vi "getFont.vi"(0 "reference":refnum<class "Graphics.lvclass">, 5 "error in (no error)":errorcluster) -> (14 "reference out":refnum<class "Graphics.lvclass">, 15 "fontType":T2=enum."Application Font", 16 "font":T1, 17 "size":i16, 19 "error out":errorcluster)   [LabVIEW 2020, in "Graphics.lvclass"]
doc: "Get font info"
uses:
  <resource>/Framework/Providers/Open_GDS/UML/Graphics_class/Graphics.lvclass
  <resource>/Framework/Providers/Open_GDS/UML/Graphics_class/LvFontType.ctl
  <resource>/Framework/Providers/Open_GDS/UML/Graphics_class/FontType.ctl
panel:
  # "Always set\nVI Server class\nto current VI. Do not\nconnect this control\nto the connector pane.\n(Tip!: Just drag\nand drop the icon\ninto the refnum)"
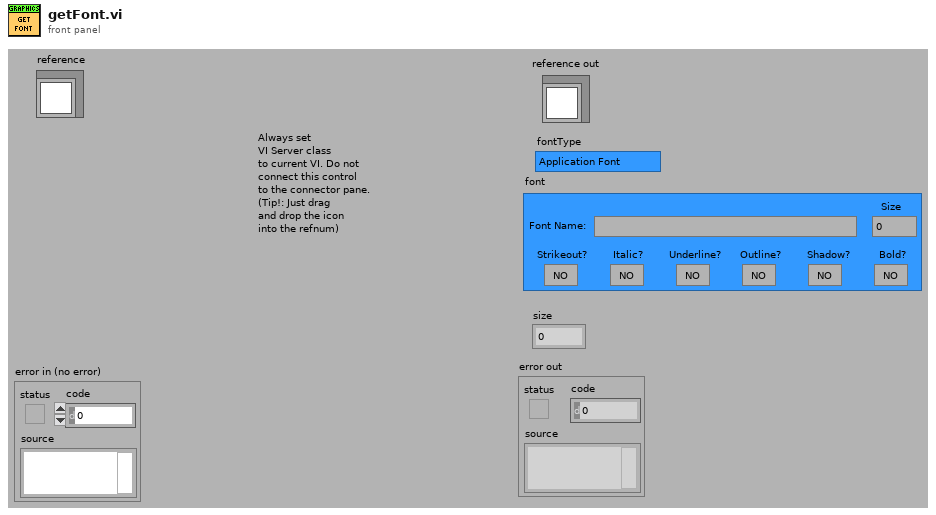
[diagram p1: front panel]
types:
  T1 = typedef "Graphics.lvclass/FontType.ctl" = cluster{"Font Name:":string, "Size":i16, "Strikeout?":bool, "Italic?":bool, "Underline?":bool, "Outline?":bool, "Shadow?":bool, "Bold?":bool}
  T2 = typedef "Graphics.lvclass/LvFontType.ctl" = enum16{"User-specified Font", "Application Font", "System Font", "Dialog Font"}
  T3 = typedef "Graphics.lvclass/ObjectAttributes.ctl" = cluster{"drawColor":u32, "backgroundColor":u32, "font":T1, "fontType":T2, "picture":picture, "stroke":T4, "scaleX":dbl, "scaleY":dbl, "screenRef":refnum<vi>, "offsetX":dbl, "offsetY":dbl}
  T4 = typedef "Graphics.lvclass/StrokeType.ctl" = enum16{"USE_DEFAULT", "SOLID", "DOTTED"}
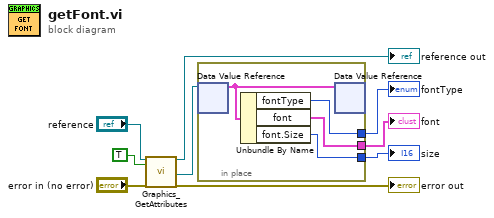
[diagram p0: block diagram]
diagram:
  n1 = call <resource>:"Graphics_GetAttributes.vi"("reference in"="reference", "OnlyGetDvrReference(False)"=TRUE, "error in (no error)"="error in (no error)") -> ("reference out"=→"reference out":refnum<class "Graphics.lvclass">, "DataRef"=w1:refnum<data-value>, "error out"=→"error out":errorcluster)  [unwired: 14 out]
  n2 = in-place {
    in-place-border: [w13] -> w5
    in-place-border: [w12] -> w4
    in-place-border: [w11] -> w3
    n3 = in-place-dvr #1(w1) -> (w10:T3)  [unwired: 1 out]
    n4 = Unbundle By Name(w10) -> ("fontType"=w13:T2, "font"=w12:T1, "font.Size"=w11:i16)
    n5 = in-place-dvr #1(w10) -> ()  [unwired: 2 out]
  }
  "size" <- w3
  "font" <- w4
  "fontType" <- w5
